vi "try to parse timestamp string.vi"(11 "possible timestamp string":string) -> (2 "valid":bool, 3 "time":timestamp)   [LabVIEW 2020, in "nominal teststand model sequence support.lvlib"]
doc: "parses timestamp by swapping date and time order, and then we pick the version that worked or if both worked we pick the one that consumed more of the string\nthat is, either of these must work:\n12:07:19 PM 7/30/2026\n7/30/2026 12:07:19 PM"
uses:
  nominal teststand model sequence support.lvlib
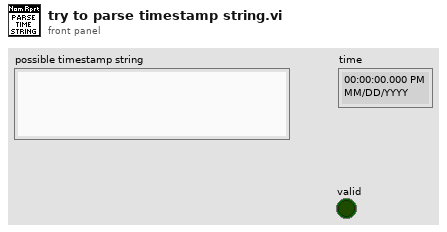
[diagram p1: front panel]
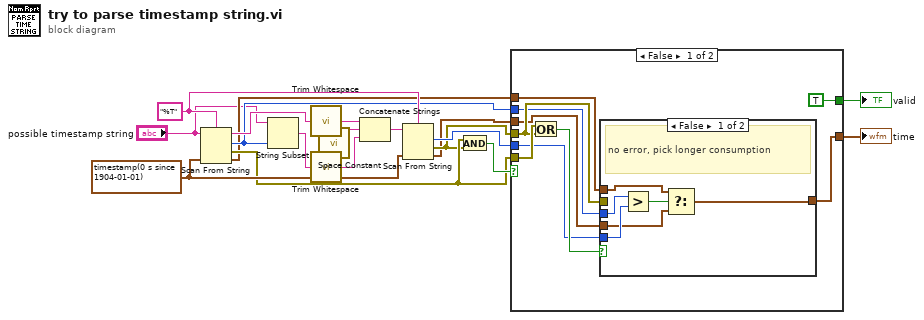
[diagram p0: block diagram]
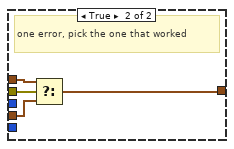
[diagram p2: hidden frame]
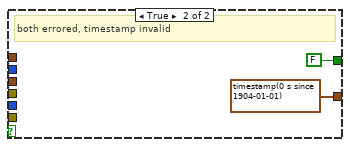
[diagram p3: hidden frame]
diagram:
  w15 = "%T" ("format string")
  w16 = timestamp(0 s since 1904-01-01)
  n1 = Scan From String(format string=w15, input string="possible timestamp string", default 1=w16) -> (remaining string=w18:string, offset past scan=w8:u32, error out=w5:errorcluster, output 1=w3:timestamp)  [unwired: 2 in]
  n2 = String Subset(string="possible timestamp string", length (rest)=w8) -> (substring=w17:string)  [unwired: 1 in]
  n3 = call <vilib>:"Trim Whitespace.vi"("string"=w18) -> ("trimmed string"=w12:string)  [unwired: 1 in]
  n4 = call <vilib>:"Trim Whitespace.vi"("string"=w17) -> ("trimmed string"=w11:string)  [unwired: 1 in]
  n5 = call <vilib>:"Space Constant.vi"() -> ("String"=w13:string)
  n6 = Concatenate Strings(w12, w13, w11) -> (w14:string)
  n7 = Scan From String(format string=w15, input string=w14, default 1=w16) -> (offset past scan=w7:u32, error out=w4:errorcluster, output 1=w2:timestamp)  [unwired: 2 in, 1 out]
  n8 = And(x=w5, y=w4) -> (x .and. y?=w10:bool)
  n9 = case shown="False" w10 {
    tunnel: [TRUE FALSE] -> w9
    tunnel: w8 -> [w20 _]
    tunnel: w7 -> [w19 _]
    tunnel: [w21 timestamp(0 s since 1904-01-01)] -> w6
    tunnel: w5 -> [w26 _]
    tunnel: w4 -> [w23 _]
    tunnel: w3 -> [w24 _]
    tunnel: w2 -> [w22 _]
    frame False {
      n10 = Or(x=w26, y=w23) -> (x .or. y?=w25:bool)
      n11 = case shown="False" w25 {
        tunnel: w24 -> [w31 w37]
        tunnel: w23 -> [_ w36]
        tunnel: w22 -> [w28 w35]
        tunnel: [w30 w34] -> w21
        tunnel: w20 -> [w33 _]
        tunnel: w19 -> [w29 _]
        frame False {
          # "no error, pick longer consumption"
          n12 = Greater?(x=w33, y=w29) -> (0:w32:bool)
          n13 = Select(t=w31, s=w32, f=w28) -> (s? t:f=w30:timestamp)
        }
        frame True {
          # "one error, pick the one that worked"
          n14 = Select(t=w37, s=w36, f=w35) -> (s? t:f=w34:timestamp)
        }
      }
    }
    frame True {
      # "both errored, timestamp invalid"
    }
  }
  "time" <- w6
  "valid" <- w9
